vi "Send Tag SetRequest_ByRef_LockBypass.vi"(4 "Timeout (-1)":i32=-1, 5 "Source (anonymous)":string="anonymous", 6 "Synchronous (F)":bool, 8 "error in (no error)":errorcluster, 9 "Value":variant, 10 "Tag Ref in":refnum<data-value>) -> (0 "error out":errorcluster, 1 "timed out?":bool, 2 "Tag Ref out":refnum<data-value>)   [LabVIEW 2020, in "Tag Engine.lvlib"]
doc: "Same as Send Tag SetRequest_ByRef, but ignores locks: the SetRequest is sent even if the Tag is locked.\n\nIntended for code that needs to set a locked Tag, such as the lock owner."
uses:
  Tag Engine.lvlib
  Tag/Tag.lvclass
  Tag/Tag.lvclass/Tag.ctl
  <vilib>/Utility/error.llb/Error Cluster From Error Code.vi
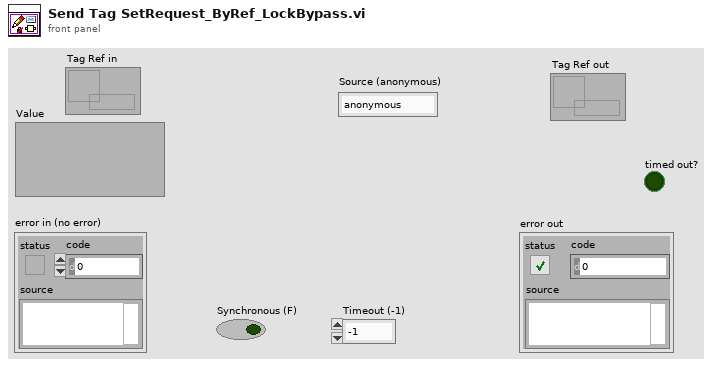
[diagram p1: front panel]
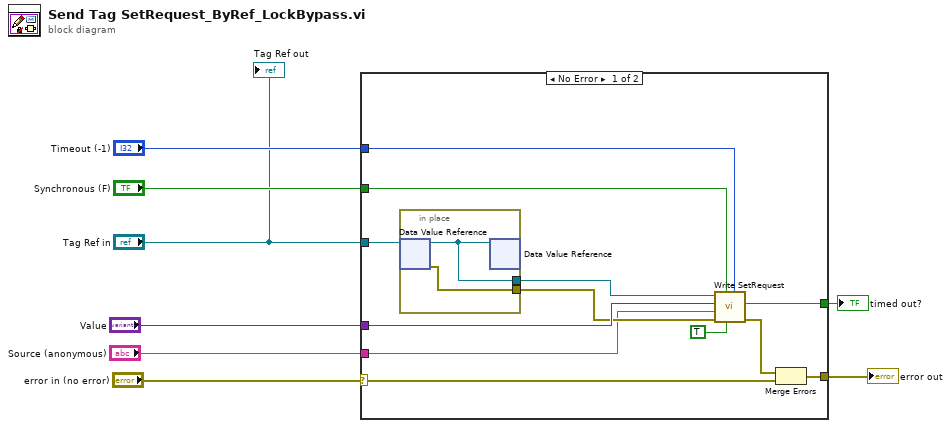
[diagram p0: block diagram]
diagram:
  n1 = case shown="No Error" "error in (no error)" {
    selector: "error in (no error)" -> [w19 w23]
    tunnel: "Tag Ref in" -> [w20 _]
    tunnel: [w18 w23] -> w8
    tunnel: "Value" -> [w17 _]
    tunnel: "Synchronous (F)" -> [w16 _]
    tunnel: "Timeout (-1)" -> [w15 _]
    tunnel: [w12 _] -> w5
    tunnel: "Source (anonymous)" -> [w9 _]
    frame No Error {
      n2 = in-place {
        in-place-border: [w22] -> w14
        in-place-border: [w21] -> w11
        n3 = in-place-dvr #1(w20) -> (w21:refnum<class "Tag.lvclass">, w22:errorcluster)
        n4 = in-place-dvr #1(w21) -> ()  [unwired: 2 out]
      }
      n5 = call "Write SetRequest.vi"("Timeout (-1)"=w15, "Ignore Lock (F)"=TRUE, "Synchronous (F)"=w16, "error in (no error)"=w14, "Source (anonymous)"=w9, "Value"=w17, "Tag in"=w11) -> ("error out"=w13:errorcluster, "timed out?"=w12:bool)  [unwired: 1 in, 2 out]
      n6 = Merge Errors(w13, w19) -> (w18:errorcluster)
    }
    frame Error {
    }
  }
  "error out" <- w8
  "timed out?" <- w5
  "Tag Ref out" <- "Tag Ref in"
